vi "Revert_TopLevelVI.vi"(8 "error in (no error)":errorcluster, 11 "Top Level/Always Included VIs":path[](array[path])) -> (0 "error out":errorcluster)   [LabVIEW 2027, in "Build VIs.lvlib"]
uses:
  Build VIs.lvlib
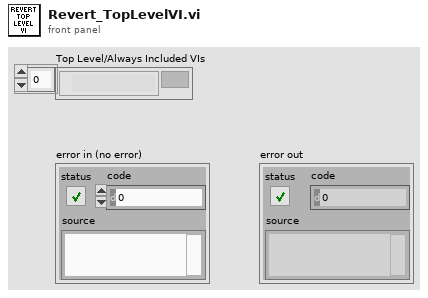
[diagram p1: front panel]
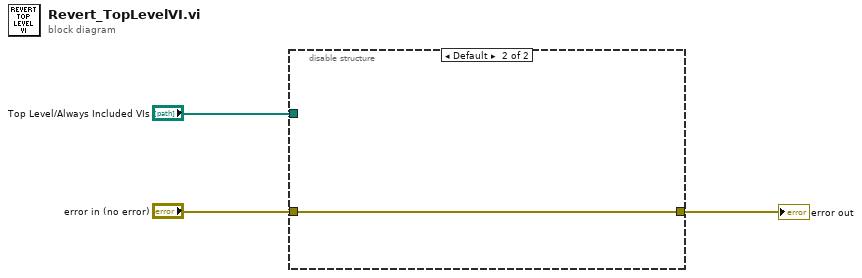
[diagram p0: block diagram]
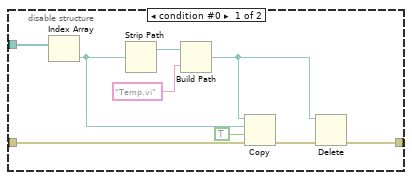
[diagram p2: hidden frame]
diagram:
  n1 = disable-structure shown="Default" {
    disable-tunnel: [w11 w13] -> w3
    disable-tunnel: "error in (no error)" -> [w9 w13]
    disable-tunnel: "Top Level/Always Included VIs" -> [w8 _]
    frame condition #0 {
      n2 = Index Array(array=w8) -> (element=w6:path)  [unwired: 1 in]
      n3 = Strip Path(path=w6) -> (stripped path=w4:path)  [unwired: 1 out]
      n4 = Build Path(base path=w4, name or relative path="Temp.vi" ("Class Name")) -> (appended path=w12:path)
      n5 = Copy(8:w9, 9:TRUE ("overwrite (F)"), 10:w6, 11:w12) -> (0:w10:errorcluster)  [unwired: 1 in, 2 out]
      n6 = Delete(path (use dialog)=w12, error in=w10) -> (error out=w11:errorcluster)  [unwired: 3 in, 2 out]
    }
    frame condition #1 (active) {
    }
  }
  "error out" <- w3
